vi "from string.vi"(8 "error in":errorcluster, 9 "data":string, 10 "version":string, 11 "engine configuration in":refnum<class "engine configuration.lvclass">) -> (0 "error out":errorcluster, 3 "engine configuration out":refnum<class "engine configuration.lvclass">)   [LabVIEW 2014, in "engine configuration.lvclass"]
doc: "Takes a version and data string and unflattens the data back into an Engine Configuration object."
uses:
  engine configuration.lvclass
  <vilib>/NI/Tag Bus/table/mapping specification.ctl
  <vilib>/NI/Tag Bus/tag/Data Type.ctl
  <vilib>/NI/Tag Bus/table/mapping.ctl
  <vilib>/NI/Tag Bus/tag/tag descriptor.lvclass
  module channel pairings.ctl
  engine configuration.lvclass/engine configuration.ctl
  <vilib>/NI/Tag Bus Module Framework/root configuration/TBM configuration.lvclass
  <vilib>/NI/Tag Bus/table/data table.lvlib
  <vilib>/NI/Configuration Framework/serializable configuration/NISE_CEF_serializable configuration.lvclass
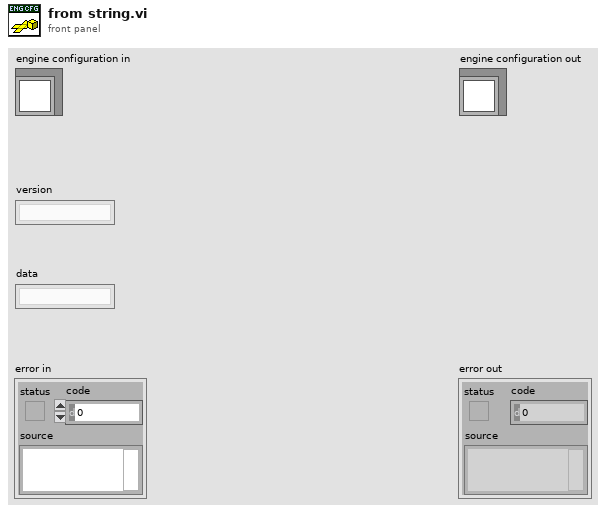
[diagram p1: front panel]
types:
  T1 = typedef "engine configuration.lvclass/module channel pairings.ctl" = cluster{"modules":string[], "channels":string[]}
  T2 = cluster{"Tag":refnum<class "tag descriptor.lvclass">, "Writer":string, "Readers":string[], "Owning ID":string}[]
  T3 = typedef "tag bus.lvlib/data table.lvlib/mapping specification.ctl" = cluster{"data type":T4, "mappings":T5[]}
  T4 = typedef "tag bus.lvlib/tag descriptor.lvclass/Data Type.ctl" = enum16{"Double", "Single", "I64", "I32", "I16", "I8", "U64", "U32", "U16", "U8", "Boolean", "String", "Array of Double", "Array of Single", "Array of I64", "Array of I32", "Array of I16", "Array of I8", "Array of U64", "Array of U32", "Array of U16", "Array of U8", "Array of Boolean", "Array of String"}
  T5 = typedef "tag bus.lvlib/data table.lvlib/mapping.ctl" = cluster{"sink name":string, "source name":string}
  T6 = cluster{"Owning ID":string, "Input Mappings":T3[], "Process Parameter Mappings":T3[], "Process Results Mappings":T3[], "Output Mappings":T3[]}[]
  T7 = cluster{"modules":string[], "channels":string[]}[]
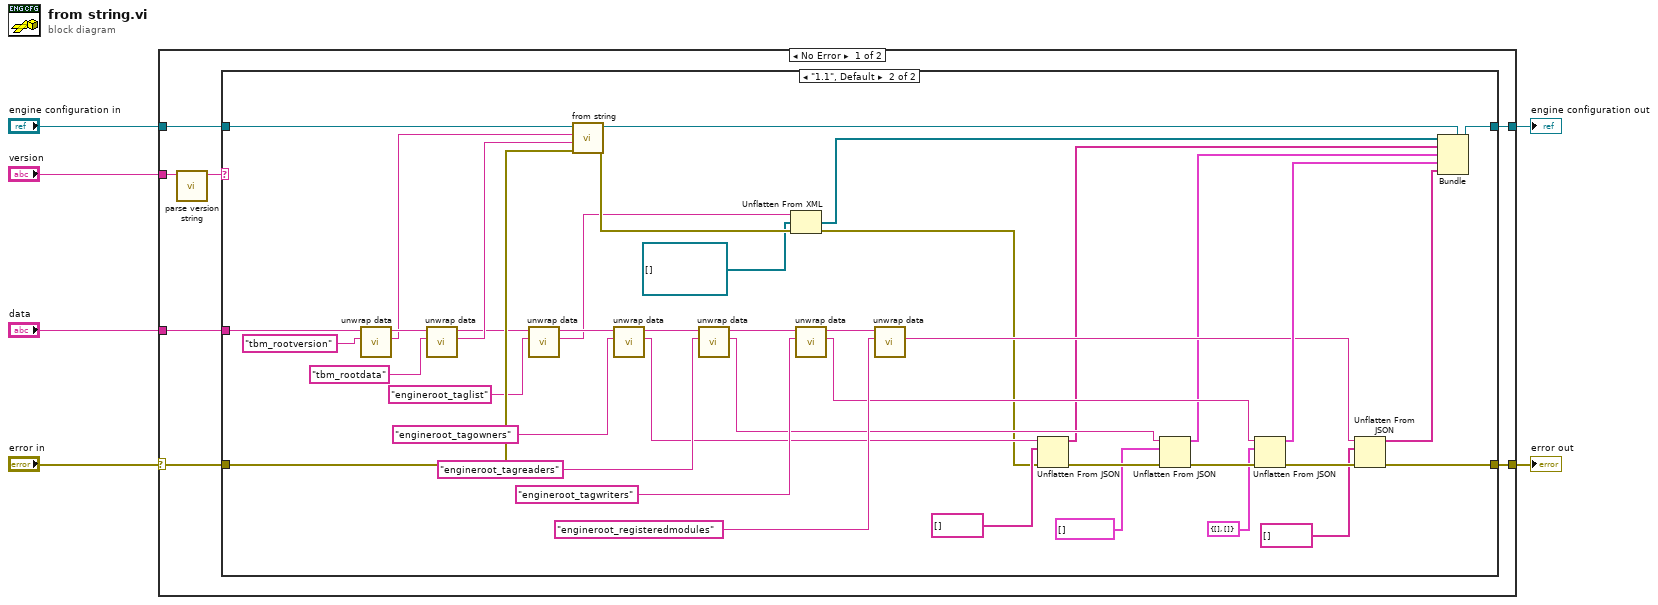
[diagram p0: block diagram]
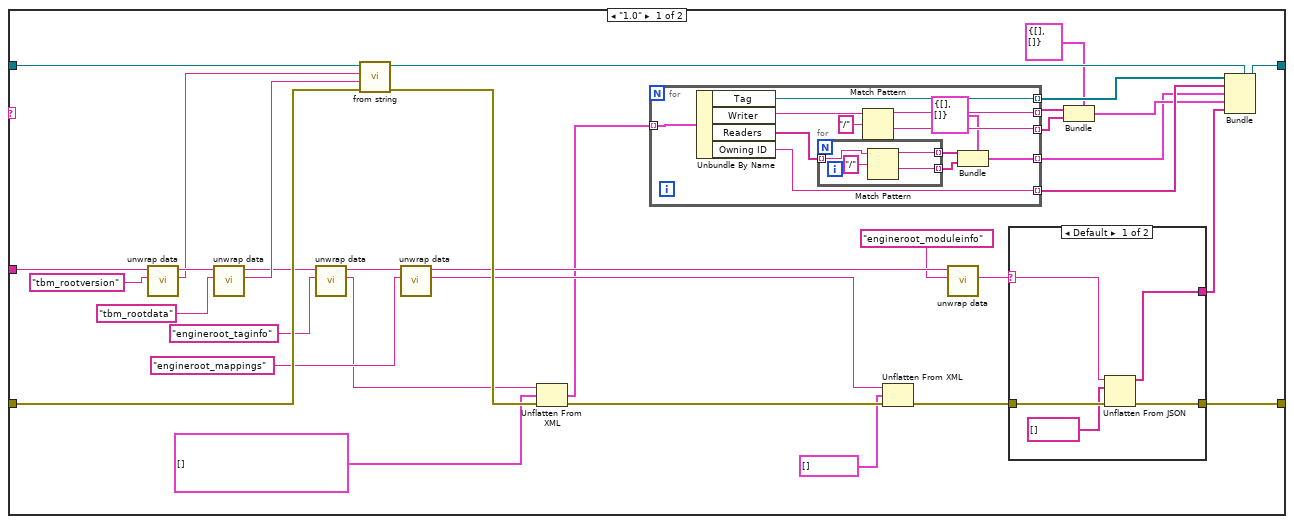
[diagram p2: hidden frame]
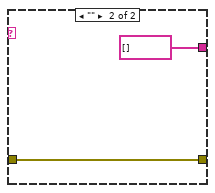
[diagram p3: hidden frame]
diagram:
  n1 = case shown="No Error" "error in" {
    selector: "error in" -> [w7 w113]
    tunnel: "data" -> [w13 _]
    tunnel: "engine configuration in" -> [w12 w112]
    tunnel: [w11 w112] -> w4
    tunnel: [w10 w113] -> w3
    tunnel: "version" -> [w9 _]
    frame No Error {
      n2 = call <vilib>:"parse version string.vi"("full version"=w9) -> ("major.minor version"=w8:string)  [unwired: 7 in, 3 out]
      n3 = case shown="\"1.1\", Default" w8 {
        tunnel: w7 -> [w47 w111]
        tunnel: w13 -> [w40 w105]
        tunnel: w12 -> [w46 w110]
        tunnel: [w36 w101] -> w11
        tunnel: [w23 w96] -> w10
        frame "1.0" {
          n4 = call <vilib>:"unwrap data.vi"("identifier"="tbm_rootversion" ("additional identifier"), "data to unwrap"=w40) -> ("unwrapped data"=w39:string, "remaining string"=w43:string)  [unwired: 8 in]
          n5 = call <vilib>:"unwrap data.vi"("identifier"="tbm_rootdata" ("additional identifier"), "data to unwrap"=w43) -> ("unwrapped data"=w38:string, "remaining string"=w33:string)  [unwired: 8 in]
          n6 = call <vilib>:"unwrap data.vi"("identifier"="engineroot_taginfo" ("additional identifier"), "data to unwrap"=w33) -> ("unwrapped data"=w28:string, "remaining string"=w32:string)  [unwired: 8 in]
          n7 = call-parent "from string.vi"("error in"=w47, "data"=w38, "version"=w39, "configuration in"=w46) -> ("error out"=w44:errorcluster, "configuration out"=w45:refnum<class "engine configuration.lvclass">)  [unwired: 6 in]
          n8 = call <vilib>:"unwrap data.vi"("identifier"="engineroot_mappings" ("additional identifier"), "data to unwrap"=w32) -> ("unwrapped data"=w29:string, "remaining string"=w27:string)  [unwired: 8 in]
          n9 = Unflatten From XML(xml string=w28, type=T2 [] ("Tag List"), error in (no error)=w44) -> (value=w21:T2, error out=w37:errorcluster)
          n10 = for {
            tunnel: w21 -> [w59] mode=indexing
            tunnel: [w56] -> w20 mode=indexing
            tunnel: [w55] -> w19 mode=indexing
            tunnel: [w54] -> w17 mode=indexing
            tunnel: [w52] -> w16 mode=indexing
            tunnel: [w48] -> w14 mode=indexing
            n11 = Unbundle By Name(w59) -> ("Tag"=w55:refnum<class "tag descriptor.lvclass">, "Writer"=w58:string, "Readers"=w53:string[], "Owning ID"=w56:string)
            n12 = for {
              tunnel: w53 -> [w62] mode=indexing
              tunnel: [w61] -> w51 mode=indexing
              tunnel: [w60] -> w50 mode=indexing
              n13 = Match Pattern(string=w62, regular expression="/") -> (before substring=w61:string, after substring=w60:string)  [unwired: 1 in, 2 out]
            }
            n14 = Match Pattern(string=w58, regular expression="/") -> (before substring=w54:string, after substring=w52:string)  [unwired: 1 in, 2 out]
            n15 = Bundle(cluster=T1 {"modules"=[], "channels"=[]} ("writers"), "modules"=w51, "channels"=w50) -> (w48:T1)
          }
          n16 = Unflatten From XML(xml string=w29, type=T6 [] ("module Mappings"), error in (no error)=w37) -> (error out=w25:errorcluster)  [unwired: 1 out]
          n17 = call <vilib>:"unwrap data.vi"("identifier"="engineroot_moduleinfo" ("additional identifier"), "data to unwrap"=w27) -> ("unwrapped data"=w24:string)  [unwired: 8 in, 1 out]
          n18 = case shown="Default" w24 {
            selector: w24 -> [w65 _]
            tunnel: w25 -> [w68 w69]
            tunnel: [w64 string[] [] ("registered modules")] -> w22
            tunnel: [w67 w69] -> w23
            frame Default {
              n19 = Unflatten From JSON(JSON string=w65, type and defaults=string[] [] ("registered modules"), error in (no error)=w68) -> (value=w64:string[], error out=w67:errorcluster)  [unwired: 4 in]
            }
            frame "" {
            }
          }
          n20 = Bundle(cluster=T1 {"modules"=[], "channels"=[]} ("writers"), "modules"=w17, "channels"=w16) -> (w15:T1)
          n21 = Bundle(cluster=w45, w19, w20, w14, w15, w22) -> (w36:refnum<class "engine configuration.lvclass">)
        }
        frame "1.1", Default {
          n22 = call <vilib>:"unwrap data.vi"("identifier"="tbm_rootversion" ("additional identifier"), "data to unwrap"=w105) -> ("unwrapped data"=w104:string, "remaining string"=w108:string)  [unwired: 8 in]
          n23 = call <vilib>:"unwrap data.vi"("identifier"="tbm_rootdata" ("additional identifier"), "data to unwrap"=w108) -> ("unwrapped data"=w103:string, "remaining string"=w100:string)  [unwired: 8 in]
          n24 = call <vilib>:"unwrap data.vi"("identifier"="engineroot_taglist" ("additional identifier"), "data to unwrap"=w100) -> ("unwrapped data"=w73:string, "remaining string"=w99:string)  [unwired: 8 in]
          n25 = call-parent "from string.vi"("error in"=w111, "data"=w103, "version"=w104, "configuration in"=w110) -> ("error out"=w75:errorcluster, "configuration out"=w109:refnum<class "engine configuration.lvclass">)  [unwired: 6 in]
          n26 = call <vilib>:"unwrap data.vi"("identifier"="engineroot_tagowners" ("additional identifier"), "data to unwrap"=w99) -> ("unwrapped data"=w81:string, "remaining string"=w92:string)  [unwired: 8 in]
          n27 = call <vilib>:"unwrap data.vi"("identifier"="engineroot_tagreaders" ("additional identifier"), "data to unwrap"=w92) -> ("unwrapped data"=w82:string, "remaining string"=w93:string)  [unwired: 8 in]
          n28 = Unflatten From XML(xml string=w73, type=refnum<class "tag descriptor.lvclass">[] [] ("tags"), error in (no error)=w75) -> (value=w71:refnum<class "tag descriptor.lvclass">[], error out=w74:errorcluster)
          n29 = call <vilib>:"unwrap data.vi"("identifier"="engineroot_tagwriters" ("additional identifier"), "data to unwrap"=w93) -> ("unwrapped data"=w84:string, "remaining string"=w94:string)  [unwired: 8 in]
          n30 = call <vilib>:"unwrap data.vi"("identifier"="engineroot_registeredmodules" ("additional identifier"), "data to unwrap"=w94) -> ("unwrapped data"=w83:string)  [unwired: 8 in, 1 out]
          n31 = Unflatten From JSON(JSON string=w81, type and defaults=string[] [] ("owners"), error in (no error)=w74) -> (value=w78:string[], error out=w102:errorcluster)  [unwired: 4 in]
          n32 = Unflatten From JSON(JSON string=w82, type and defaults=T7 [] ("readers"), error in (no error)=w102) -> (value=w77:T7, error out=w97:errorcluster)  [unwired: 4 in]
          n33 = Unflatten From JSON(JSON string=w84, type and defaults=cluster{"modules":string[], "channels":string[]} {"modules"=[], "channels"=[]} ("writers"), error in (no error)=w97) -> (value=w85:cluster{"modules":string[], "channels":string[]}, error out=w95:errorcluster)  [unwired: 4 in]
          n34 = Unflatten From JSON(JSON string=w83, type and defaults=string[] [] ("registered modules"), error in (no error)=w95) -> (value=w76:string[], error out=w96:errorcluster)  [unwired: 4 in]
          n35 = Bundle(cluster=w109, w71, w78, w77, w85, w76) -> (w101:refnum<class "engine configuration.lvclass">)
        }
      }
    }
    frame Error {
    }
  }
  "error out" <- w3
  "engine configuration out" <- w4
